vi "RemoteVI Capture Windows.vi"(0 "windows":T2(array[cluster])) -> (4 "captures":T1(array[cluster]))   [LabVIEW 2020, in "RemoteVI.lvlib"]
doc: "Captures every listed window (docs\\protocol.md section 7) the way the main frame is captured: RemoteVI Capture Frame.vi on its HWND - PrintWindow, cut to the client area, no VI Server call, so it works while a dialog's modal loop holds LabVIEW's UI thread (measured on LabVIEW 2025 for a Two Button Dialog and a native file dialog). A window that could not be drawn gives an empty pixmap with width and height 0; RemoteVI Send Window Frame.vi sends nothing for it. Order follows windows."
uses:
  RemoteVI.lvlib
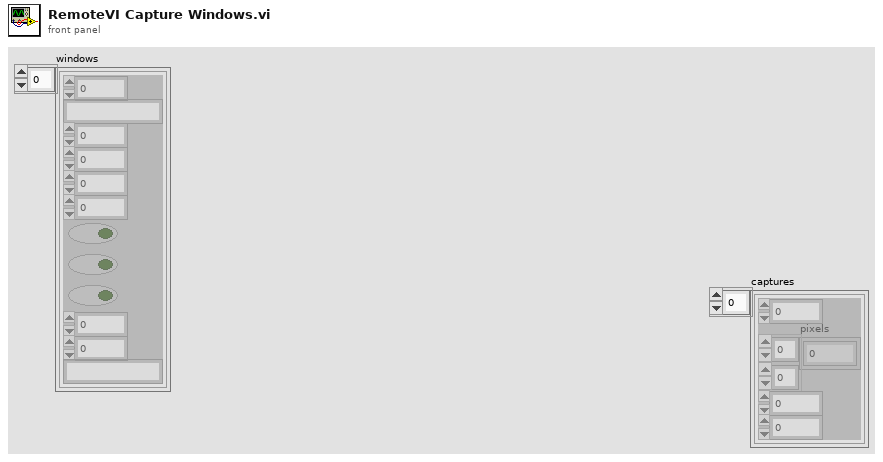
[diagram p1: front panel]
types:
  T1 = cluster{"id":u64, "pixels":u32[][], "width":i32, "height":i32}[]
  T2 = cluster{"id":u64, "title":string, "x":i32, "y":i32, "w":i32, "h":i32, "modal":bool, "active":bool, "closable":bool, "sx":i32, "sy":i32, "class":string}[]
  T3 = cluster{"id":u64, "pixels":u32[][], "width":i32, "height":i32}
  T4 = cluster{"pixmap":u32[][], "width":i32, "height":i32, "time":u32}
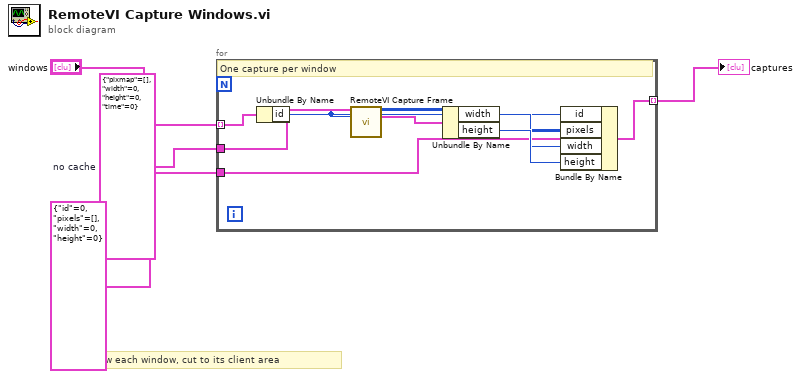
[diagram p0: block diagram]
diagram:
  w2 = T4 {"pixmap"=[], "width"=0, "height"=0, "time"=0}  # no cache
  # "PrintWindow each window, cut to its client area"
  n1 = for {
    tunnel: "windows" -> [w5] mode=indexing
    tunnel: w2 -> [w6]
    tunnel: T3 {"id"=0, "pixels"=[], "width"=0, "height"=0} -> [w7]
    tunnel: [w13] -> w4 mode=indexing
    # "One capture per window"
    n2 = Unbundle By Name(w5) -> ("id"=w8:u64)
    n3 = call "RemoteVI Capture Frame.vi"("cache"=w6, "hWnd"=w8) -> ("frame"=w9:u32[][], "cache out"=w10:T4)  [unwired: 12 in]
    n4 = Unbundle By Name(w10) -> ("width"=w11:i32, "height"=w12:i32)
    n5 = Bundle By Name(cluster=w7, "id"=w8, "pixels"=w9, "width"=w11, "height"=w12) -> (w13:T3)
  }
  "captures" <- w4
